vi "Close Log File.vi"(8 "error in (no error)":errorcluster, 11 "Log File":refnum<k34>) -> (0 "error out":errorcluster)   [LabVIEW 2016]
uses:
  <vilib>/WebDAVClient/Simple Put File.vi
  <vilib>/WebDAVClient/NI_WebDAV.lvlib
panel:
  out "Error out WebDAV Put @ cRIO":errorcluster
  # "Após todas as amostras serem armazenadas no arquivo, o mesmo é fechado e o arquivo de indexação excluído.\nDetalhes sobre a transferência via WebDAV estão no diagrama de blocos"
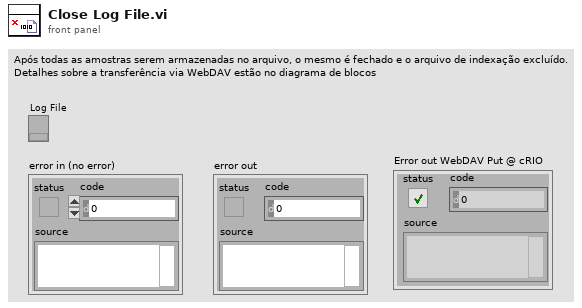
[diagram p1: front panel]
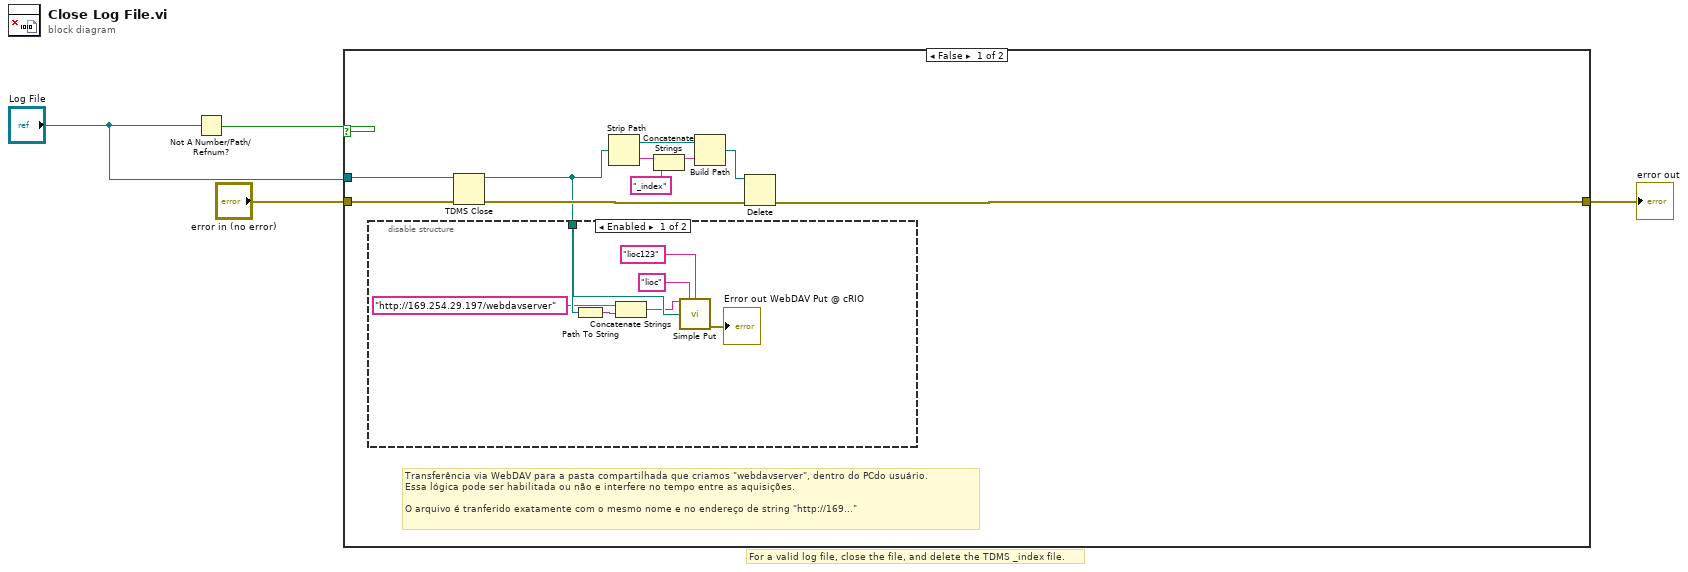
[diagram p0: block diagram]
diagram:
  # "For a valid log file, close the file, and delete the TDMS _index file."
  n1 = Not A Number/Path/Refnum?(number/path/refnum="Log File") -> (NaN/Path/Refnum?=w1:bool)
  n2 = case shown="False" w1 {
    tunnel: [w14 w22] -> w4
    tunnel: "error in (no error)" -> [w13 w22]
    tunnel: "Log File" -> [w12 _]
    frame False {
      # "Transferência via WebDAV para a pasta compartilhada que criamos \"webdavserver\", dentro do PCdo usuário.\nEssa lógica pode ser habilitada ou não e interfere no tempo entre as aquisições.\n\nO arquivo é tranferido exatamente com o mesmo nome e no endereço de string \"http://169...\""
      n3 = TDMS Close(8:w13, 11:w12) -> (0:w6:errorcluster, 3:w5:path)
      n4 = disable-structure shown="Enabled" {
        disable-tunnel: w5 -> [w21 _]
        frame Enabled {
          n5 = Path To String(path=w21) -> (string=w17:string)
          n6 = Concatenate Strings("http://169.254.29.197/webdavserver", w17) -> (w15:string)
          n7 = call-poly <vilib>:"Simple Put.vi"("file uri"=w15, "username"="lioc", "password"="lioc123", "local file path"=w21) -> ("error out"=→"Error out WebDAV Put @ cRIO":errorcluster)  [unwired: 10 in, 1 out]
        }
        frame Disabled {
        }
      }
      n8 = Strip Path(path=w5) -> (stripped path=w9:path, name=w7:string)
      n9 = Concatenate Strings(w7, "_index") -> (w10:string)
      n10 = Build Path(base path=w9, name or relative path=w10) -> (appended path=w11:path)
      n11 = Delete(path (use dialog)=w11, error in=w6) -> (error out=w14:errorcluster)  [unwired: 3 in, 2 out]
    }
    frame True {
    }
  }
  "error out" <- w4
